vi "FindWindowExW Wrapper Template.vi"(0 "hWndParent":u64, 5 "hWndChildAfter":u64, 7 "lpszClass":u16[](array[numeric]), 9 "lpszWindow":u16[](array[numeric]), 11 "error in":errorcluster) -> (4 "hWnd":u64, 15 "error out":errorcluster)   [LabVIEW 2020]
doc: "Finds a window through user32.dll FindWindowExW (stdcall, called in any thread): the next child of hWndParent after hWndChildAfter in Z order whose class and title match. With hWndParent 0 it walks the TOP-LEVEL windows, so calling it repeatedly with the previous answer as hWndChildAfter enumerates them without a callback. lpszClass and lpszWindow are UTF-16 code units WITH a terminating 0; an EMPTY array passes NULL, which matches any class or title. hWnd is 0 when no further window matches. When error in carries an error the DLL is not called. Generated by tools\\Build Win32 Wrappers.vi - do not edit by hand, rebuild it."
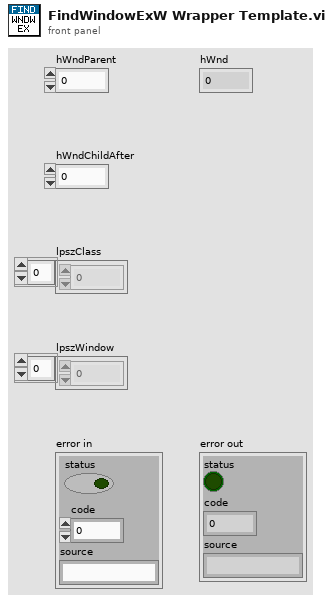
[diagram p1: front panel]
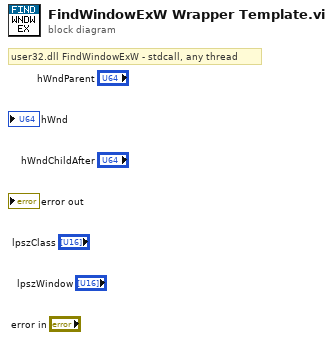
[diagram p0: block diagram]
diagram:
  # "user32.dll FindWindowExW - stdcall, any thread"
